vi "Do Core.vi"(8 "error in (no error)":errorcluster, 9 "Actor in":refnum<class "Actor.lvclass">, 11 "Reply Message":refnum<class "Get Minimum Trigger Interval Msg.lvclass">) -> (0 "error out":errorcluster, 1 "Actor out":refnum<class "Actor.lvclass">, 2 "Reply":variant)   [LabVIEW 2020, in "DAQ Timed SPIM.lvlib" / "Abstract DAQ Triggered Actor.lvlib" / "Get Minimum Trigger Interval Msg.lvclass"]
doc: "(<B>Filename</B>: Actor Framework.lvlib:Reply Msg.lvclass:Do Core.vi)\n\nDefines what an actor does when it receives <B>Reply Message</B>. This method also defines the <B>Reply</B> that is returned to the actor that sent <B>Reply Message</B>.\n\nBy default, this method does nothing, and <B>Reply</B> is the ancestor Message class. A child class must override this method to define behavior and specify a child of the Message class to return in the <B>Reply</B> output."
uses:
  Get Minimum Trigger Interval Msg.lvclass
  <vilib>/ActorFramework/Actor/Actor.lvclass
  Abstract DAQ Triggered Actor/Abstract DAQ Triggered Actor.lvclass
  C:/Program Files/National Instruments/LabVIEW 2020/vi.lib/ActorFramework/Actor/Actor.lvclass
  1f71038e-5174-4cbf-9fd5-6f0c7527817e.vi
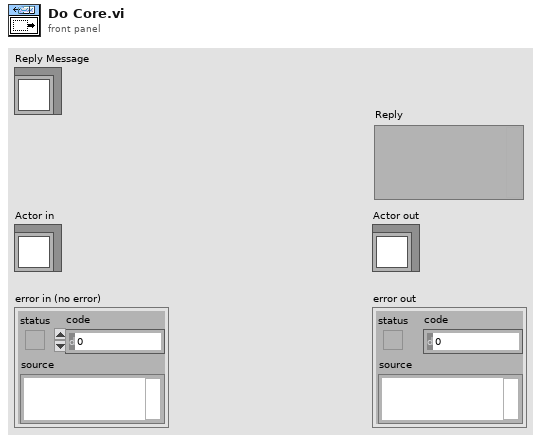
[diagram p1: front panel]
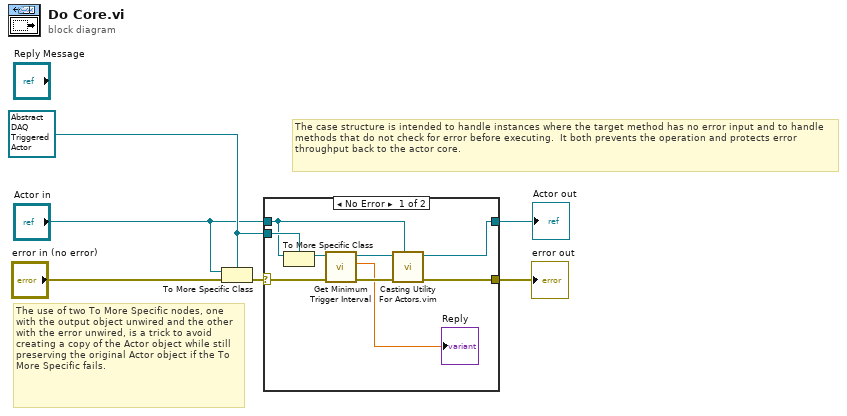
[diagram p0: block diagram]
diagram:
  w5 = refnum<class "Abstract DAQ Triggered Actor.lvclass"> refnum ("Actor in")
  # "The use of two To More Specific nodes, one with the output object unwired and the other with the error unwired, is a trick to avoid creating a copy of the Actor object while still preserving the original Actor object if the To More Specific fails."
  # "The case structure is intended to handle instances where the target method has no error input and to handle methods that do not check for error before executing.  It both prevents the operation and protects error throughput back to the actor core."
  n1 = To More Specific Class(target class=w5, reference="Actor in", error in="error in (no error)") -> (error out=w6:errorcluster)  [unwired: 1 out]
  n2 = case shown="No Error" w6 {
    selector: w6 -> [w15 w17]
    tunnel: [w9 w17] -> w3
    tunnel: [w10 w16] -> w2
    tunnel: "Actor in" -> [w12 w16]
    tunnel: w5 -> [w13 _]
    frame No Error {
      n3 = To More Specific Class(target class=w13, reference=w12) -> (specific class reference=w14:refnum<class "Abstract DAQ Triggered Actor.lvclass">)  [unwired: 1 in, 1 out]
      n4 = call-dynamic "Get Minimum Trigger Interval.vi"("error in (no error)"=w15, "Abstract DAQ Triggered Actor in"=w14) -> ("error out"=w8:errorcluster, "Minimum Interval (ms)"=→"Reply":dbl, "Abstract DAQ Triggered Actor out"=w11:refnum<class "Abstract DAQ Triggered Actor.lvclass">)  [unwired: 7 in]
      n5 = call "Casting Utility For Actors.vim"("type"=w12, "error in (no error)"=w8, "Actor in"=w11) -> ("error out"=w9:errorcluster, "Actor out"=w10:refnum<class "Actor.lvclass">)  [unwired: 7 in]
    }
    frame Error {
      # "If type check fails, pass the original object out again."
    }
  }
  "error out" <- w3
  "Actor out" <- w2
